vi "UMLEditor Main.vi"(1 "StartProject":string, 3 "StartTarget":string) -> ()   [LabVIEW 2020] (continued)
            n1299 = call <resource>:"CommonVIs SterotypeStringParser.vi"("SterotypeStringIn"=w3426) -> ("Name"=w3422:string)  [unwired: 18 out]
            n1300 = Search 1D Array(1D array=w3423, element=w3422) -> (index of element=w3421:i32)  [unwired: 1 out]
            n1301 = Less Than 0?(x=w3421) -> (x < 0?=w3418:bool)
            n1302 = case shown="False" w3418 {
              selector: w3418 -> [_ w3466]
              tunnel: [w3462 w3466] -> w3417
              frame False {
                n1303 = Two Button Dialog(message="There is already on object on the diagram with this name.\nDo you want to add this object anyway?" ("regular expression"), 1:"Cancel" ("regular expression"), 2:"Add object" ("regular expression")) -> (T button?=w3462:bool)
              }
              frame True {
              }
            }
            n1304 = Compound Arithmetic op=AND(TRUE, w3437, w3435, w3417) -> (w3436:bool)
            n1305 = case shown="False" w3436 {
              tunnel: w3461 -> [w3478 w3515]
              tunnel: [w3478 w3514] -> w3460
              tunnel: w3424 -> [w3470 w3513]
              tunnel: w3427 -> [w3471 w3512]
              tunnel: [w3477 w3507] -> w3458
              tunnel: [w3469 w3506] -> w3457
              tunnel: w3426 -> [_ w3505]
              tunnel: w3453 -> [w3467 w3504]
              tunnel: w3451 -> [_ w3502]
              tunnel: w3428 -> [_ w3503]
              tunnel: w3420 -> [w3476 _]
              tunnel: w3419 -> [w3468 _]
              frame False {
                n1306 = call <vilib>:"Check if File or Folder Exists.vi"("path"=w3467) -> ("file or folder exists?"=w3473:bool)  [unwired: 1 in, 9 out]
                n1307 = Equal?(x=T27 "StateDiagramGraph" ("diagramType"), y=w3476) -> (x = y?=w3474:bool)
                n1308 = And(x=w3474, y=w3473) -> (x .and. y?=w3472:bool)
                n1309 = case shown="True" w3472 {
                  tunnel: [UMLEditor_statesType."Idle" ("state") UMLEditor_statesType."Repaint" ("state")] -> w3477
                  tunnel: w3471 -> [_ w3485]
                  tunnel: w3470 -> [w3479 w3483]
                  tunnel: [w3479 w3491] -> w3469
                  tunnel: w3468 -> [_ w3489]
                  tunnel: w3467 -> [_ w3486]
                  frame False {
                  }
                  frame True {
                    n1310 = To More Specific Class(target class=refnum<class "StateDiagramGraph.lvclass"> refnum ("reference out"), reference=w3485, error in=w3483) -> (specific class reference=w3484:refnum<class "StateDiagramGraph.lvclass">, error out=w3482:errorcluster)
                    n1311 = Unbundle By Name(w3489) -> ("graphics"=w3488:refnum<class "Graphics.lvclass">, "grid"=w3487:refnum<class "Grid.lvclass">)
                    n1312 = call <resource>:"SetPathInfo.vi"("reference"=w3484, "StateDiagramData.VI-Path"=w3486, "error in (no error)"=w3482) -> ("reference out"=w3493:refnum<class "StateDiagramGraph.lvclass">, "error out"=w3492:errorcluster)  [unwired: 1 in, 14 out]
                    n1313 = call-dynamic "HandleRightClickMenuOption.vi"("reference"=w3493, "MenuOption"="Update diagram...", "graphics"=w3488, "grid"=w3487, "error in (no error)"=w3492) -> ("error out"=w3491:errorcluster)  [unwired: 12 in, 2 out]
                  }
                }
              }
              frame True {
                n1314 = call-dynamic "findNode.vi"("reference"=w3512, "error in (no error)"=w3513) -> ("reference out"=w3499:refnum<class "Graph.lvclass">, "node"=w3511:refnum<class "AbstractNode.lvclass">, "found"=w3510:bool, "error out"=w3497:errorcluster)  [unwired: 14 in]
                n1315 = call <resource>:"ClassNode_Create.vi"("error in (no error)"=w3497) -> ("reference out"=w3495:refnum<class "ClassNode.lvclass">, "error out"=w3496:errorcluster)  [unwired: 17 in]
                n1316 = call <resource>:"FindFreePosition.vi"("reference"=w3499, "NodePointIn"=w3502, "Node"=w3495, "error in (no error)"=w3496) -> ("reference out"=w3498:refnum<class "Graph.lvclass">, "NodePointOut"=w3501:T9, "error out"=w3500:errorcluster)  [unwired: 13 out]
                n1317 = call-dynamic "add.vi"("reference"=w3498, "node"=w3495, "point"=w3501, "error in (no error)"=w3500) -> ("added"=w3509:bool, "error out"=w3508:errorcluster)  [unwired: 13 in, 1 out]
                n1318 = case shown="True" w3509 {
                  tunnel: w3515 -> [w3525 w3556]
                  tunnel: [w3524 w3554] -> w3514
                  tunnel: w3508 -> [w3520 w3551]
                  tunnel: w3495 -> [w3518 w3540]
                  tunnel: w3501 -> [w3522 w3552]
                  tunnel: [w3521 w3557] -> w3506
                  tunnel: w3510 -> [w3517 _]
                  tunnel: w3511 -> [w3523 _]
                  tunnel: w3505 -> [_ w3549]
                  tunnel: [UMLEditor_statesType."Idle" ("state") w3548] -> w3507
                  tunnel: w3504 -> [_ w3542]
                  tunnel: w3503 -> [_ w3541]
                  frame False {
                    n1319 = call-dynamic "Destroy.vi"("reference"=w3518, "error in (no error)"=w3520) -> ("error out"=w3519:errorcluster)  [unwired: 16 in, 1 out]
                    n1320 = case shown="True" w3517 {
                      tunnel: w3525 -> [w3526 w3539]
                      tunnel: [w3526 w3538] -> w3524
                      tunnel: w3523 -> [_ w3537]
                      tunnel: w3522 -> [_ w3536]
                      tunnel: [w3527 w3535] -> w3521
                      tunnel: w3519 -> [w3527 w3534]
                      frame False {
                      }
                      frame True {
                        # "Node Found"
                        n1321 = call-dynamic "getBounds.vi"("reference"=w3537, "error in (no error)"=w3534) -> ("bounds"=w3532:T10, "error out"=w3535:errorcluster)  [unwired: 15 in, 1 out]
                        n1322 = Build Array(w3537) -> (w3531:refnum<class "AbstractNode.lvclass">[])
                        n1323 = Bundle By Name(cluster=w3539, "selected"=UMLEditor_tooltype."Node" ("selcted"), "SelectedNodes"=w3531, "dragStartBounds"=w3532, "dragStartPoint"=w3536, "lastMousePoint"=w3536, "newSelected"=TRUE, "toolType"=UMLEditor_tooltype."None") -> (w3538:T5)
                        n1324 = local write "GraphButtons"(T1."1" ("GraphButtons")) -> ()
                      }
                    }
                  }
                  frame True {
                    # "Added"
                    n1325 = case shown="\"AddNodeFromProjectTree+SyncAll\"" w3541 {
                      tunnel: [UMLEditor_statesType."Repaint" ("state") UMLEditor_statesType."SyncAll" ("state")] -> w3548
                      frame "AddNodeFromProjectTree", Default {
                      }
                      frame "AddNodeFromProjectTree+SyncAll" {
                      }
                    }
                    n1326 = call-dynamic "ExternalSetParam.vi"("reference"=w3540, "setParameter"=ExternalSetTypes."Name", "string"=w3549, "error in (no error)"=w3551) -> ("reference out"=w3545:refnum<class "ClassNode.lvclass">, "error out"=w3547:errorcluster)  [unwired: 14 in]
                    n1327 = call-dynamic "ExternalSetParam.vi"("reference"=w3545, "setParameter"=ExternalSetTypes."ClassPath", "error in (no error)"=w3547, "ClassPath"=w3542) -> ("reference out"=w3544:refnum<class "ClassNode.lvclass">, "error out"=w3546:errorcluster)  [unwired: 14 in]
                    n1328 = call-dynamic "getBounds.vi"("reference"=w3544, "error in (no error)"=w3546) -> ("reference out"=w3561:refnum<class "ClassNode.lvclass">, "bounds"=w3562:T10, "error out"=w3558:errorcluster)  [unwired: 15 in]
                    n1329 = Build Array(w3561) -> (w3553:refnum<class "ClassNode.lvclass">[])
                    n1330 = Bundle By Name(cluster=w3556, "selected"=UMLEditor_tooltype."Node" ("selcted"), "SelectedNodes"=w3553, "dragStartBounds"=w3562, "dragStartPoint"=w3552, "lastMousePoint"=w3552) -> (w3555:T5)
                    n1331 = call <resource>:"UMLEditor setDiagramInfo.vi"("error in (no error)"=w3558, "localVariablesIn"=w3555, "action"=enum16{"Name/Dir", "Unsaved", "Saved"}."Unsaved") -> ("localVariablesOut"=w3554:T5, "error out"=w3557:errorcluster)  [unwired: 2 in, 13 out]
                  }
                }
              }
            }
            n1332 = for {
              tunnel: w3457 -> [_]
              tunnel: w3432 -> [w3577] mode=indexing
              tunnel: [w3576] -> _
              n1333 = Close Reference(reference=w3577) -> (error out=w3576:errorcluster)  [unwired: 1 in]
            }
          }
          frame True {
            n1334 = call <resource>:"GDSError_ClearError.vi"("code"=1055, "error in (no error)"=w3580) -> ("error out"=w3579:errorcluster)  [unwired: 3 in, 14 out]
          }
        }
      }
      frame "AnalyseViInStateDiagram" {
        n1335 = Unbundle By Name(w3589) -> ("diagrams"=w3610:T8[])
        n1336 = Unbundle By Name(w3589) -> ("menu"=w3604:refnum<k9>, "Action"=w3588:string)
        n1337 = property on="GraphButtons" class="RadioBtnsControl (strict)"("Disabled"=u8 0) -> ()  [unwired: 2 in, 2 out]
        n1338 = local write "Diagram"(0) -> ()
        n1339 = local write "GraphButtons"(T1."1" ("GraphButtons")) -> ()
        n1340 = for {
          tunnel: w3610 -> [w3654] mode=indexing
          tunnel: "Untitled %d" -> [w3652]
          tunnel: [w3651] -> w3608 mode=indexing
          n1341 = Unbundle By Name(w3654) -> ("name"=w3653:string)
          n1342 = Scan From String(format string=w3652, input string=w3653) -> (output 1=w3651:i32)  [unwired: 2 in, 4 out]
        }
        n1343 = String To Path(string=w3588) -> (path=w3587:path)
        n1344 = Bundle By Name(cluster=T29 {"VI-Path"=path "", "ShowOption"=enum."Show Relative Path"} ("StateDiagramData"), "VI-Path"=w3587) -> (w3594:T29)
        n1345 = Unbundle By Name(w3589) -> ("grid"=w3596:refnum<class "Grid.lvclass">, "graphics"=w3595:refnum<class "Graphics.lvclass">)
        n1346 = Array Max & Min(array=w3608) -> (max value=w3607:i32)  [unwired: 3 out]
        n1347 = call <resource>:"StateDiagramGraph_Create.vi"("StateDiagramData"=w3594, "error in (no error)"=w3593) -> ("reference out"=w3599:refnum<class "StateDiagramGraph.lvclass">, "error out"=w3598:errorcluster)  [unwired: 1 in, 15 out]
        n1348 = property on="Picture" class="Pict"() -> (error out=w3586:errorcluster, "Visible"=w3585:bool)  [unwired: 2 in, 1 out]
        n1349 = call-dynamic "HandleRightClickMenuOption.vi"("reference"=w3599, "MenuOption"="Create New Diagram", "graphics"=w3595, "grid"=w3596, "error in (no error)"=w3598) -> ("reference out"=w3592:refnum<class "StateDiagramGraph.lvclass">, "Cancel"=w3591:bool, "error out"=w3590:errorcluster)  [unwired: 12 in]
        n1350 = property on="Picture" class="Pict"(error in=w3586, "Visible"=TRUE) -> ()  [unwired: 1 in, 2 out]
        n1351 = case shown="False" w3591 {
          tunnel: w3607 -> [w3636 _]
          tunnel: w3604 -> [w3623 _]
          tunnel: [w3622 w3648] -> w3603
          tunnel: [w3621 w3647] -> w3602
          tunnel: w3589 -> [w3620 w3647]
          tunnel: [UMLEditor_statesType."Repaint" ("state") UMLEditor_statesType."Idle" ("state")] -> w3601
          tunnel: w3592 -> [w3618 w3649]
          tunnel: w3590 -> [w3617 w3650]
          tunnel: w3585 -> [_ w3645]
          frame False {
            n1352 = local read "Help"() -> (w3613:bool)
            n1353 = call <resource>:"UndoEngine.vi"("Reference In"=w3618, "Action"=enum16{"TakeSnapshot", "Undo", "Redo"}."TakeSnapshot", "Reset"=TRUE, "error in (no error)"=w3617, "menu"=w3623) -> ("Reference Out"=w3615:refnum<class "StateDiagramGraph.lvclass">, "error out"=w3612:errorcluster)  [unwired: 3 in, 10 out]
            n1354 = case shown="True" w3613 {
              tunnel: w3615 -> [w3639 w3644]
              tunnel: [w3639 w3643] -> w3614
              tunnel: [w3638 w3642] -> w3611
              tunnel: w3612 -> [w3638 w3641]
              frame False {
              }
              frame True {
                n1355 = call-dynamic "GetDiagramHelpText.vi"("reference in"=w3644, "error in (no error)"=w3641) -> ("reference out"=w3643:refnum<class "StateDiagramGraph.lvclass">, "HelpOut"=w3640:T38, "error out"=w3642:errorcluster)  [unwired: 15 in]
                n1356 = call <resource>:"ContextHelp_SendMessageToPopUp.vi"("PopUpMessage"=w3640) -> ()  [unwired: 2 in, 17 out]
              }
            }
            n1357 = Increment(x=w3636) -> (x+1=w3634:i32)
            n1358 = Format Into String(format string="Untitled %d", w3634) -> (resulting string=w3631:string)  [unwired: 2 in, 1 out]
            n1359 = property on="Diagram" class="Ring (strict)"("Tip Strip"=w3631) -> ()  [unwired: 2 in, 2 out]
            n1360 = call <resource>:"UMLEditor addDiagram.vi"("graph"=w3614, "name"=w3631, "saveDir"=path "", "unsaved(False)"=FALSE, "error in (no error)"=w3611, "localVariablesIn"=w3620) -> ("localVariablesOut"=w3616:T5, "error out"=w3632:errorcluster)  [unwired: 1 in, 11 out]
            n1361 = Unbundle By Name(w3620) -> ("menu"=w3629:refnum<k9>)
            n1362 = Bundle By Name(cluster=w3616, "selectedEdge"=refnum<class "AbstractEdge.lvclass"> refnum, "SelectedNodes"=refnum<class "AbstractNode.lvclass">[] [], "selected"=UMLEditor_tooltype."None" ("selcted")) -> (w3621:T5)
            n1363 = call <resource>:"UMLEditor menuUpdates.vi"("menu"=w3629, "menuAction"=UMLEditor_MenuActionType."EnableSave", "error in (no error)"=w3632) -> ("error out"=w3622:errorcluster)  [unwired: 3 in, 13 out]
          }
          frame True {
            n1364 = property on="Picture" class="Pict"("Visible"=w3645) -> ()  [unwired: 2 in, 2 out]
            n1365 = call-dynamic "Destroy.vi"("reference"=w3649, "error in (no error)"=w3650) -> ("error out"=w3648:errorcluster)  [unwired: 17 in]
          }
        }
      }
      frame "Copy", "CopyPaste" {
        n1366 = Unbundle By Name(w3656) -> ("SelectedNodes"=w3657:refnum<class "AbstractNode.lvclass">[], "menu"=w3660:refnum<k9>)
        n1367 = Array Size(array=w3657) -> (size(s)=w3661:i32)
        n1368 = case shown="1.." w3661 {
          tunnel: w3660 -> [_ w3677]
          tunnel: w3659 -> [w3665 w3669]
          tunnel: [w3665 w3670] -> w3658
          tunnel: w3657 -> [_ w3671]
          tunnel: w3656 -> [_ w3666]
          frame 0, Default {
          }
          frame 1.. {
            n1369 = call <resource>:"UMLEditor getDiagramInfo.vi"("localVariables"=w3666, "error in (no error)"=w3669) -> ("graph"=w3667:refnum<class "Graph.lvclass">, "error out"=w3668:errorcluster)  [unwired: 16 out]
            n1370 = call <resource>:"UMLEditor menuUpdates.vi"("menu"=w3677, "menuAction"=UMLEditor_MenuActionType."EnablePaste", "error in (no error)"=w3668) -> ("error out"=w3675:errorcluster)  [unwired: 3 in, 13 out]
            n1371 = call <resource>:"UMLEditor ClipBoard.vi"("menuAction"=UMLEditor_ClipBoardActionType."EmptyClipBoard", "error in (no error)"=w3675) -> ("error out"=w3673:errorcluster)  [unwired: 4 in, 13 out]
            n1372 = call <resource>:"UMLEditor ClipBoard.vi"("menuAction"=UMLEditor_ClipBoardActionType."InsertToClipBoard", "SelectedNodes"=w3671, "Graph"=w3667, "error in (no error)"=w3673) -> ("error out"=w3670:errorcluster)  [unwired: 2 in, 13 out]
          }
        }
        n1373 = case shown="\"CopyPaste\"" w3655 {
          tunnel: [UMLEditor_statesType."Paste" ("state") UMLEditor_statesType."Idle" ("state")] -> w3662
          frame "CopyPaste" {
          }
          frame Default {
          }
        }
      }
      frame "Paste" {
        n1374 = Unbundle By Name(w3679) -> ("graphics"=w3684:refnum<class "Graphics.lvclass">, "offset"=w3686:T9, "zoom"=w3685:dbl)
        n1375 = call <resource>:"UMLEditor getDiagramInfo.vi"("localVariables"=w3679, "error in (no error)"=w3683) -> ("graph"=w3680:refnum<class "Graph.lvclass">, "diagramType"=w3681:T27, "error out"=w3682:errorcluster)  [unwired: 15 out]
        n1376 = case shown="Default" w3681 {
          tunnel: [w3690 w3712] -> w3687
          tunnel: w3686 -> [_ w3709]
          tunnel: w3685 -> [_ w3708]
          tunnel: w3684 -> [_ w3707]
          tunnel: w3682 -> [w3690 w3699]
          tunnel: w3680 -> [_ w3698]
          tunnel: w3679 -> [w3689 w3697]
          tunnel: [w3689 w3696] -> w3678
          frame "", "None" {
          }
          frame Default {
            w3706 = cluster{dbl, dbl} {0.0, 0.0} ("lower limit")
            n1377 = property on="Picture" class="Pict"() -> ("Mouse"=w3701:T41)  [unwired: 2 in, 2 out]
            n1378 = Unbundle By Name(w3701) -> ("Mouse Position"=w3711:cluster{"X":i32, "Y":i32})
            n1379 = Add(x=w3711, y=w3709) -> (x+y=w3710:T9)
            n1380 = Divide(x=w3710, y=w3708) -> (x/y=w3692:T9)
            n1381 = call <resource>:"getScreenBounds.vi"("reference"=w3707, "error in (no error)"=w3699) -> ("bounds"=w3705:T10, "error out"=w3700:errorcluster)  [unwired: 16 out]
            n1382 = Unbundle By Name(w3705) -> ("width"=w3704:dbl, "height"=w3703:dbl)
            n1383 = Bundle(cluster=w3706, w3704, w3703) -> ()  [unwired: 1 out]
            n1384 = In Range and Coerce(upper limit=w3692, x=w3692, lower limit=w3706) -> (coerced(x)=w3702:T9)  [unwired: 1 out]
            n1385 = call <resource>:"UMLEditor ClipBoard.vi"("menuAction"=UMLEditor_ClipBoardActionType."PasteContentAtPos", "Pos"=w3702, "Graph"=w3698, "error in (no error)"=w3700, "LimitPasteToAllowedLocations(True)"=FALSE) -> ("PastedNodes"=w3695:refnum<class "AbstractNode.lvclass">[], "error out"=w3712:errorcluster)  [unwired: 2 in, 11 out]
            n1386 = Array Size(array=w3695) -> (size(s)=w3693:i32)
            n1387 = case shown="0" w3693 {
              tunnel: [UMLEditor_tooltype."Node" ("selcted") UMLEditor_tooltype."None" ("selcted")] -> w3694
              frame Default {
              }
              frame 0 {
              }
            }
            n1388 = Bundle By Name(cluster=w3697, "selected"=w3694, "SelectedNodes"=w3695) -> (w3696:T5)
          }
        }
      }
      frame "Export" {
        w3717 = 0.0 ("y")
        w3716 = 5.0  # borderRoundPicture
        w3751 = 1.0 ("scaleX")
        n1389 = Unbundle By Name(w3724) -> ("graphics"=w3754:refnum<class "Graphics.lvclass">)
        n1390 = Unbundle By Name(w3724) -> ("exportype"=w3723:T11)
        n1391 = Unbundle By Name(w3724) -> ("grid"=w3746:refnum<class "Grid.lvclass">)
        n1392 = call-dynamic "clone.vi"("reference"=w3754, "error in (no error)"=w3753) -> ("clonedObjectRef"=w3752:refnum<class "Graphics.lvclass">, "error out"=w3750:errorcluster)  [unwired: 15 in, 1 out]
        n1393 = call <resource>:"scale.vi"("reference"=w3752, "scaleX"=w3751, "scaleY"=w3751, "error in (no error)"=w3750) -> ("reference out"=w3742:refnum<class "Graphics.lvclass">, "error out"=w3743:errorcluster)  [unwired: 14 out]
        n1394 = call <resource>:"resetPicture.vi"("reference"=w3742, "error in (no error)"=w3743) -> ("reference out"=w3741:refnum<class "Graphics.lvclass">, "error out"=w3740:errorcluster)  [unwired: 16 out]
        n1395 = call <resource>:"UMLEditor getDiagramInfo.vi"("localVariables"=w3724, "error in (no error)"=w3740) -> ("graph"=w3748:refnum<class "Graph.lvclass">, "name"=w3721:string, "saveDir"=w3722:path, "error out"=w3749:errorcluster)  [unwired: 14 out]
        n1396 = call-dynamic "getBounds.vi"("reference"=w3748, "graphics"=w3741, "error in (no error)"=w3749) -> ("reference out"=w3747:refnum<class "Graph.lvclass">, "bounds"=w3734:T10, "error out"=w3739:errorcluster)  [unwired: 14 in]
        n1397 = Unbundle By Name(w3734) -> ("width"=w3732:dbl, "height"=w3733:dbl)
        n1398 = Unbundle By Name(w3734) -> ("x"=w3738:dbl, "y"=w3735:dbl)
        n1399 = Subtract(x=w3738, y=w3717) -> (x-y=w3737:dbl)
        n1400 = Subtract(x=w3735, y=w3717) -> (x-y=w3736:dbl)
        n1401 = Add(x=w3732, y=w3733) -> (x+y=w3731:dbl)
        n1402 = Greater Than 0?(x=w3731) -> (x > 0?=w3730:bool)
        n1403 = call <resource>:"setOffset.vi"("reference"=w3741, "offsetX"=w3737, "offsetY"=w3736, "error in (no error)"=w3739) -> ("reference out"=w3729:refnum<class "Graphics.lvclass">, "error out"=w3718:errorcluster)  [unwired: 14 out]
        n1404 = Multiply(x=w3716, y=2.0) -> (x*y=w3725:dbl)
        n1405 = call-dynamic "draw.vi"("reference"=w3747, "graphics"=w3729, "grid"=w3746, "error in (no error)"=w3718, "SelectedNodes"=refnum<class "AbstractNode.lvclass">[] [], "HideOverLays(False)"=TRUE) -> ("NodesBounds"=w3745:T10, "error out"=w3727:errorcluster)  [unwired: 10 in, 2 out]
        n1406 = case shown="True" w3730 {
          tunnel: w3745 -> [_ _]
          tunnel: w3734 -> [_ w3778]
          tunnel: w3729 -> [_ w3779]
          tunnel: w3727 -> [w3756 w3764]
          tunnel: [w3756 w3764] -> w3728
          tunnel: w3725 -> [_ w3768]
          tunnel: w3723 -> [_ w3763]
          tunnel: w3723 -> [_ w3771]
          tunnel: w3722 -> [_ w3770]
          tunnel: w3721 -> [_ w3765]
          tunnel: w3716 -> [_ w3758]
          frame False {
          }
          frame True {
            n1407 = Match Pattern(string=w3765, regular expression="[.][~.]+$") -> (before substring=w3766:string)  [unwired: 4 out]
            n1408 = Unbundle By Name(w3778) -> ("x"=w3761:dbl, "y"=w3759:dbl, "width"=w3776:dbl, "height"=w3774:dbl)
            n1409 = case shown="\"jpg\"" w3771 {
              tunnel: w3770 -> [_ w3787 w3792 _]
              tunnel: w3766 -> [_ w3785 w3790 _]
              tunnel: [path "" ("Not A Path Constant") w3783 w3788 path "" ("Not A Path Constant")] -> w3769
              frame "None", Default {
              }
              frame "png" {
                n1410 = Concatenate Strings(w3785, ".png" ("string")) -> (w3786:string)
                n1411 = Build Path(base path=w3787, name or relative path=w3786) -> (appended path=w3783:path)
              }
              frame "jpg" {
                n1412 = Concatenate Strings(w3790, ".jpg" ("string")) -> (w3791:string)
                n1413 = Build Path(base path=w3792, name or relative path=w3791) -> (appended path=w3788:path)
              }
              frame "Printer" {
              }
            }
            n1414 = Subtract(x=w3761, y=w3758) -> (x-y=w3760:dbl)
            n1415 = Subtract(x=w3759, y=w3758) -> (x-y=w3757:dbl)
            n1416 = Add(x=w3776, y=w3768) -> (x+y=w3775:dbl)
            n1417 = Add(x=w3774, y=w3768) -> (x+y=w3773:dbl)
            n1418 = Bundle By Name(cluster=T10 {"x"=0.0, "y"=0.0, "width"=0.0, "height"=0.0} ("bounds"), "x"=w3760, "y"=w3757, "width"=w3775, "height"=w3773) -> (w3772:T10)
            n1419 = call <resource>:"UMLEditor export.vi"("graphics"=w3779, "bounds"=w3772, "exportype"=w3763, "fileName"=w3769, "error in (no error)"=w3764) -> ("error out"=w3762:errorcluster)  [unwired: 14 out]
            n1420 = case shown="\"Printer\"" w3763 {
              tunnel: w3762 -> [_ w3780]
              frame "None", Default {
              }
              frame "Printer" {
                n1421 = case shown="Error" w3780 {
                  frame No Error {
                  }
                  frame Error {
                    n1422 = One Button Dialog(message="Error while printing\nCheck the default printer settings.") -> ()  [unwired: 2 out]
                  }
                }
              }
            }
          }
        }
        n1423 = call-dynamic "Destroy.vi"("reference"=w3729, "error in (no error)"=w3728) -> ("error out"=w3744:errorcluster)  [unwired: 16 in, 1 out]
      }
      frame "EditSelected" {
        n1424 = Unbundle By Name(w3796) -> ("selected"=w3807:T7, "selectedEdge"=w3801:refnum<class "AbstractEdge.lvclass">, "SelectedNodes"=w3805:refnum<class "AbstractNode.lvclass">[])
        n1425 = Unbundle By Name(w3796) -> ("graphics"=w3795:refnum<class "Graphics.lvclass">, "grid"=w3794:refnum<class "Grid.lvclass">)
        n1426 = call <resource>:"UMLEditor getDiagramInfo.vi"("localVariables"=w3796, "error in (no error)"=w3804) -> ("graph"=w3802:refnum<class "Graph.lvclass">, "diagramType"=w3799:T27, "error out"=w3803:errorcluster)  [unwired: 15 out]
        n1427 = Bundle By Name(cluster=w3796, "newSelected"=FALSE) -> (w3798:T5)
        n1428 = case shown="\"Node\"" w3807 {
          tunnel: w3803 -> [w3813 w3843 w3911]
          tunnel: [w3811 w3844 w3905] -> w3806
          tunnel: w3805 -> [_ w3832 _]
          tunnel: w3802 -> [w3812 w3839 w3909]
          tunnel: w3801 -> [_ _ w3908]
          tunnel: w3798 -> [w3810 w3830 w3907]
          tunnel: [w3809 w3834 w3906] -> w3800
          tunnel: w3799 -> [w3814 _ _]
          tunnel: w3795 -> [_ w3827 _]
          tunnel: w3794 -> [_ w3826 _]
          frame "None", Default {
            n1429 = case shown="\"StateDiagramGraph\"" w3814 {
              tunnel: w3813 -> [w3816 w3825]
              tunnel: w3812 -> [_ w3819]
              tunnel: [w3816 w3822] -> w3811
              tunnel: w3810 -> [w3815 w3821]
              tunnel: [w3815 w3820] -> w3809
              frame Default {
              }
              frame "StateDiagramGraph" {
                n1430 = To More Specific Class(target class=refnum<class "StateDiagramGraph.lvclass"> refnum ("reference out"), reference=w3819) -> (specific class reference=w3817:refnum<class "StateDiagramGraph.lvclass">)  [unwired: 1 in, 1 out]
                n1431 = call-dynamic "editDialog.vi"("reference"=w3817, "error in (no error)"=w3825) -> ("error out"=w3823:errorcluster)  [unwired: 15 in, 2 out]
                n1432 = call <resource>:"UMLEditor setDiagramInfo.vi"("error in (no error)"=w3823, "localVariablesIn"=w3821, "action"=enum16{"Name/Dir", "Unsaved", "Saved"}."Unsaved") -> ("localVariablesOut"=w3820:T5, "error out"=w3822:errorcluster)  [unwired: 2 in, 13 out]
              }
            }
          }
          frame "Node" {
            n1433 = Index Array(array=w3832) -> (element=w3829:refnum<class "AbstractNode.lvclass">)  [unwired: 1 in]
            n1434 = call-dynamic "contains.vi"("reference"=w3839, "node"=w3829, "nodeType(Empty=AllNodeTypesAllaowed)"=string[] ["PackageNode$", "SystemNode$"], "error in (no error)"=w3843) -> ("contains"=w3838:bool, "container"=w3837:refnum<class "AbstractNode.lvclass">, "error out"=w3842:errorcluster)  [unwired: 12 in, 1 out]
            n1435 = call-dynamic "editDialog.vi"("reference"=w3829, "insidePackageNode"=w3838, "error in (no error)"=w3842) -> ("reference out"=w3836:refnum<class "AbstractNode.lvclass">, "changeConnection"=w3841:T54, "cancel"=w3835:bool, "error out"=w3840:errorcluster)  [unwired: 13 in]
            n1436 = Build Array(w3829) -> (w3828:refnum<class "AbstractNode.lvclass">[])
            n1437 = Bundle By Name(cluster=w3830, "SelectedNodes"=w3828) -> (w3831:T5)
            n1438 = case shown="False" w3835 {
              tunnel: [w3851 w3903] -> w3844
              tunnel: w3841 -> [w3858 _]
              tunnel: w3840 -> [w3857 w3903]
              tunnel: w3839 -> [w3847 _]
              tunnel: w3837 -> [w3856 _]
              tunnel: w3836 -> [w3855 _]
              tunnel: w3831 -> [w3850 w3902]
              tunnel: [w3849 w3902] -> w3834
              tunnel: w3827 -> [w3846 _]
              tunnel: w3826 -> [w3845 _]
              frame False {
                n1439 = case shown="\"Connect\"" w3858 {
                  tunnel: w3857 -> [w3861 w3869 w3874]
                  tunnel: w3856 -> [_ w3868 w3895]
                  tunnel: w3855 -> [w3860 w3866 w3872]
                  tunnel: [w3861 w3863 w3886] -> w3854
                  tunnel: [w3859 _ _] -> w3848
                  tunnel: w3847 -> [_ w3862 w3890]
                  tunnel: w3846 -> [_ _ w3889]
                  tunnel: w3845 -> [_ _ w3888]
                  frame "NA", Default {
                    n1440 = Build Array(w3860) -> (w3859:refnum<class "AbstractNode.lvclass">[])
                  }
                  frame "Connect" {
                    n1441 = call-dynamic "addChild.vi"("reference"=w3868, "node"=w3866, "error in (no error)"=w3869) -> ("reference out"=w3865:refnum<class "AbstractNode.lvclass">, "error out"=w3867:errorcluster)  [unwired: 15 in]
                    n1442 = call-dynamic "setParent.vi"("reference"=w3866, "node"=w3865, "error in (no error)"=w3867) -> ("error out"=w3864:errorcluster)  [unwired: 15 in, 1 out]
                    n1443 = call-dynamic "RearrangeNodes.vi"("reference in"=w3862, "error in (no error)"=w3864) -> ("error out"=w3863:errorcluster)  [unwired: 16 in, 1 out]
                  }
                  frame "DisConnect" {
                    n1444 = call-dynamic "GetParentsRecurivly.vi"("reference"=w3872, "error in (no error)"=w3874) -> ("Parents"=w3871:refnum<class "AbstractNode.lvclass">[], "error out"=w3873:errorcluster)  [unwired: 15 in, 1 out]
                    n1445 = call-dynamic "removeChild.vi"("reference"=w3895, "node"=w3872, "error in (no error)"=w3873) -> ("reference out"=w3891:refnum<class "AbstractNode.lvclass">, "error out"=w3894:errorcluster)  [unwired: 15 in]
                    n1446 = call-dynamic "setParent.vi"("reference"=w3872, "node"=refnum<class "AbstractNode.lvclass"> refnum, "error in (no error)"=w3894) -> ("error out"=w3892:errorcluster)  [unwired: 15 in, 1 out]
                    n1447 = call-dynamic "layout.vi"("reference"=w3891, "graph"=w3890, "graphics"=w3889, "grid"=w3888, "error in (no error)"=w3892) -> ("error out"=w3887:errorcluster)  [unwired: 13 in, 1 out]
                    n1448 = Delete From Array(array=w3871) -> (deleted portion=w3870:refnum<class "AbstractNode.lvclass">)  [unwired: 2 in, 1 out]
                    n1449 = call-dynamic "getBounds.vi"("reference"=w3870, "error in (no error)"=w3887) -> ("bounds"=w3884:T10, "error out"=w3885:errorcluster)  [unwired: 15 in, 1 out]
                    n1450 = call <resource>:"Rectangel GetRectInfo.vi"("bounds"=w3884) -> ("maxX"=w3882:dbl)  [unwired: 1 in, 17 out]
                    n1451 = call-dynamic "getBounds.vi"("reference"=w3872, "error in (no error)"=w3885) -> ("reference out"=w3877:refnum<class "AbstractNode.lvclass">, "bounds"=w3883:T10, "error out"=w3876:errorcluster)  [unwired: 15 in]
                    n1452 = Unbundle By Name(w3883) -> ("x"=w3881:dbl)
                    n1453 = Subtract(x=w3882, y=w3881) -> (x-y=w3880:dbl)
                    n1454 = Add(x=10.0, y=w3880) -> (x+y=w3878:dbl)
                    n1455 = Greater Or Equal To 0?(x=w3878) -> (x >= 0?=w3875:bool)
                    n1456 = case shown="True" w3875 {
                      tunnel: [w3896 w3901] -> w3886
                      tunnel: w3878 -> [_ w3900]
                      tunnel: w3877 -> [_ w3899]
                      tunnel: w3876 -> [w3896 w3898]
                      frame False {
                      }
                      frame True {
                        n1457 = call-dynamic "translate.vi"("reference"=w3899, "dx"=w3900, "dy"=0.0, "error in (no error)"=w3898) -> ("error out"=w3901:errorcluster)  [unwired: 14 in, 1 out]
                      }
                    }
                  }
                }
                n1458 = call-dynamic "layout.vi"("reference"=w3847, "LayoutNodes(Empty=All)"=w3848, "error in (no error)"=w3854) -> ("error out"=w3852:errorcluster)  [unwired: 15 in, 1 out]
                n1459 = call <resource>:"UMLEditor setDiagramInfo.vi"("error in (no error)"=w3852, "localVariablesIn"=w3850, "action"=enum16{"Name/Dir", "Unsaved", "Saved"}."Unsaved") -> ("localVariablesOut"=w3849:T5, "error out"=w3851:errorcluster)  [unwired: 2 in, 13 out]
              }
              frame True {
              }
            }
          }
          frame "Edge" {
            n1460 = call-dynamic "editDialog.vi"("reference"=w3908, "error in (no error)"=w3911) -> ("cancel"=w3904:bool, "error out"=w3910:errorcluster)  [unwired: 15 in, 1 out]
            n1461 = case shown="True" w3904 {
              tunnel: w3910 -> [w3919 w3925]
              tunnel: w3909 -> [w3918 _]
              tunnel: w3907 -> [w3916 w3924]
              tunnel: [w3915 w3924] -> w3906
              tunnel: [w3913 w3925] -> w3905
              frame False {
                n1462 = case shown="False" FALSE ("Case Constant\n(See Context Help) 4") {
                  tunnel: w3919 -> [w3920 w3923]
                  tunnel: w3918 -> [_ w3922]
                  tunnel: [w3920 w3921] -> w3914
                  frame False {
                  }
                  frame True {
                    n1463 = call-dynamic "layout.vi"("reference"=w3922, "error in (no error)"=w3923) -> ("error out"=w3921:errorcluster)  [unwired: 16 in, 1 out]
                  }
                }
                n1464 = call <resource>:"UMLEditor setDiagramInfo.vi"("error in (no error)"=w3914, "localVariablesIn"=w3916, "action"=enum16{"Name/Dir", "Unsaved", "Saved"}."Unsaved") -> ("localVariablesOut"=w3915:T5, "error out"=w3913:errorcluster)  [unwired: 2 in, 13 out]
              }
              frame True {
              }
            }
          }
        }
      }
      frame "RemoveSelected" {
        # "if aggregartion, check if we should remove ClassRef Attribute"
        n1465 = Unbundle By Name(w3934) -> ("selected"=w3930:T7, "selectedEdge"=w3936:refnum<class "AbstractEdge.lvclass">, "SelectedNodes"=w3935:refnum<class "AbstractNode.lvclass">[], "Don'tDeleteChildren"=w3926:bool)
        n1466 = call <resource>:"UMLEditor getDiagramInfo.vi"("localVariables"=w3934, "error in (no error)"=w3938) -> ("graph"=w3937:refnum<class "Graph.lvclass">, "error out"=w3927:errorcluster)  [unwired: 16 out]
        n1467 = case shown="\"Node\"" w3930 {
          tunnel: [w3951 w3959 w3979] -> w3932
          tunnel: w3937 -> [_ w3958 w3981]
          tunnel: w3927 -> [w3951 w3956 w3978]
          tunnel: w3936 -> [_ w3957 _]
          tunnel: w3935 -> [_ _ w3980]
          tunnel: w3926 -> [_ _ w3977]
          frame "None", Default {
          }
          frame "Edge" {
            n1468 = call <resource>:"UMLEditor ShowAggregationDialog.vi"("graph"=w3958, "ClassAggregation"=w3957, "error in (no error)"=w3956) -> ("Base class.bounds"=w3953:T10, "Remove"=w3954:bool, "StartEndNodes"=w3952:T37, "error out"=w3955:errorcluster)  [unwired: 13 out]
            n1469 = stacked-sequence {
              tunnel: [w3966] -> w3959
              tunnel: w3958 -> [w3965]
              tunnel: w3957 -> [w3964]
              tunnel: w3956 -> [w3963]
              tunnel: w3955 -> [_]
              tunnel: w3954 -> [w3962]
              tunnel: w3953 -> [w3961]
              tunnel: w3952 -> [w3960]
              frame #0 {
                n1470 = case shown="True" w3962 {
                  tunnel: w3961 -> [_ w3973]
                  tunnel: w3960 -> [_ w3967]
                  frame False {
                  }
                  frame True {
                    n1471 = Unbundle(w3973) -> ("x"=w3972:dbl, "y"=w3968:dbl, "width"=w3971:dbl)  [unwired: 1 out]
                    n1472 = Add(x=w3972, y=w3971) -> (x+y=w3970:dbl)
                    n1473 = Bundle(cluster=cluster{"X":i32, "Y":i32} {"X"=100, "Y"=100} ("Mouse Position"), "X"=w3970, "Y"=w3968) -> (w3969:cluster{"X":i32, "Y":i32})
                    n1474 = call <resource>:"UMLEditor_AggregationClusterDialogControl.vi"("Position"=w3969, "Action(SelectSelect)"=T19."DeleteAggregation", "StartEndNodesIn"=w3967) -> ()  [unwired: 6 in, 11 out]
                  }
                }
                n1475 = call-dynamic "removeEdge.vi"("reference"=w3965, "edge"=w3964, "error in (no error)"=w3963) -> ("error out"=w3966:errorcluster)  [unwired: 15 in, 1 out]
              }
            }
          }
          frame "Node" {
            n1476 = Not(x=w3977) -> (.not. x?=w3976:bool)
            n1477 = for {
              tunnel: w3981 -> [w3986]
              tunnel: w3980 -> [w3985] mode=indexing
              shift-right: [w3984] -> w3979
              shift-left: w3978 -> [w3983]
              tunnel: w3976 -> [w3982]
              n1478 = call-dynamic "removeNode.vi"("reference"=w3986, "node"=w3985, "RemoveChildrenIfAny(False)"=w3982, "error in (no error)"=w3983) -> ("error out"=w3984:errorcluster)  [unwired: 14 in, 1 out]
            }
          }
        }
        n1479 = Bundle By Name(cluster=w3934, "selected"=UMLEditor_tooltype."None" ("selcted")) -> (w3929:T5)
        n1480 = case shown="\"Node\", \"Edge\"" w3930 {
          tunnel: w3932 -> [w3941 w3949]
          tunnel: [w3941 w3948] -> w3931
          tunnel: [w3940 w3945] -> w3928
          tunnel: w3929 -> [w3940 w3947]
          frame "None", Default {
          }
          frame "Node", "Edge" {
            n1481 = call <resource>:"UMLEditor setDiagramInfo.vi"("error in (no error)"=w3949, "localVariablesIn"=w3947, "action"=enum16{"Name/Dir", "Unsaved", "Saved"}."Unsaved") -> ("localVariablesOut"=w3946:T5, "error out"=w3948:errorcluster)  [unwired: 2 in, 13 out]
            n1482 = Bundle By Name(cluster=w3946, "SelectedNodes"=refnum<class "AbstractNode.lvclass">[] [], "selectedEdge"=refnum<class "AbstractEdge.lvclass"> refnum, "modified"=TRUE) -> (w3945:T5)
          }
        }
      }
      frame "Save" {
        w3990 = UMLEditor_statesType."Close" ("x")
        n1483 = Unbundle By Name(w3992) -> ("saveAs"=w3994:bool)
        n1484 = call <resource>:"UMLEditor getDiagramInfo.vi"("localVariables"=w3992, "error in (no error)"=w4013) -> ("graph"=w4011:refnum<class "Graph.lvclass">, "name"=w4004:string, "saveDir"=w4001:path, "error out"=w4010:errorcluster)  [unwired: 14 out]
        n1485 = Empty String/Path?(string/path=w4001) -> (empty?=w3989:bool)
        n1486 = File/Directory Info(path=w4001, error in=w4010) -> (directory=w3999:bool, error out=w4008:errorcluster)  [unwired: 5 out]
        n1487 = call <resource>:"File_ApplicationPaths.vi"("PathName"=UMLEditor_StoredPathes."LastSearchPath" ("UMLPathes")) -> ("Path Out"=w3987:path)  [unwired: 3 in, 15 out]
        n1488 = Bundle By Name(cluster=w3992, "saveAs"=FALSE) -> (w3993:T5)
        n1489 = Compound Arithmetic op=AND(invert w3994, invert w3989, w3999) -> (w4000:bool)
        n1490 = case shown="False" w4000 {
          tunnel: w4008 -> [w4031 w4054]
          tunnel: [w4030 w4054] -> w4007
          tunnel: [w4025 w4056] -> w4006
          tunnel: w4001 -> [w4016 w4056]
          tunnel: [w4024 w4055] -> w4005
          tunnel: w4004 -> [w4023 w4055]
          tunnel: w3993 -> [w4029 w4057]
          tunnel: [w4028 w4057] -> w4003
          tunnel: [w4019 FALSE ("cancelled")] -> w4002
          tunnel: w3989 -> [w4017 _]
          tunnel: w3987 -> [w4014 _]
          frame False {
            (unwired) T49."new or existing file" ("select mode (2)")
            n1491 = Select(t=w4014, s=w4017, f=w4016) -> (s? t:f=w4015:path)
            n1492 = File Dialog(6:"*.uml" ("pattern"), 7:"Select file name" ("prompt"), 11:w4015) -> (1:w4020:bool, 2:w4022:bool, 3:w4021:path)  [unwired: 1 in, 4 out]
            n1493 = case shown="True" w4022 {
              tunnel: [w4032 w4035] -> w4019
              tunnel: w4020 -> [w4032 _]
              tunnel: w4021 -> [w4033 w4034]
              tunnel: [w4033 w4034] -> w4018
              frame False {
              }
              frame True {
                n1494 = Two Button Dialog(message="This file already exists.\nDo you want to overwrite it?", 1:"No" ("F button name (\"Cancel\")"), 2:"Yes" ("T button name (\"OK\")")) -> (T button?=w4036:bool)
                n1495 = case shown="True" w4036 {
                  tunnel: w4034 -> [_ w4040]
                  frame False {
                  }
                  frame True {
                    n1496 = Delete(path (use dialog)=w4040) -> ()  [unwired: 1 in, 6 out]
                  }
                }
                n1497 = Not(x=w4036) -> (.not. x?=w4035:bool)
              }
            }
            n1498 = case shown="False" w4019 {
              tunnel: w4031 -> [w4047 w4049]
              tunnel: [w4046 w4049] -> w4030
              tunnel: w4029 -> [w4045 w4052]
              tunnel: [w4044 w4052] -> w4028
              tunnel: w4018 -> [w4043 _]
              tunnel: [w4042 w4051] -> w4025
              tunnel: [w4041 w4050] -> w4024
              tunnel: w4015 -> [_ w4051]
              tunnel: w4023 -> [_ w4050]
              frame False {
                n1499 = Strip Path(path=w4043) -> (stripped path=w4042:path, name=w4041:string)
                n1500 = call <resource>:"UMLEditor setDiagramInfo.vi"("name"=w4041, "saveDir"=w4042, "error in (no error)"=w4047, "localVariablesIn"=w4045, "action"=enum16{"Name/Dir", "Unsaved", "Saved"}."Name/Dir") -> ("localVariablesOut"=w4044:T5, "error out"=w4046:errorcluster)  [unwired: 13 out]
              }
              frame True {
              }
            }
          }
          frame True {
          }
        }
        n1501 = Equal?(x=w3990, y=w3998) -> (x = y?=w3997:bool)
        n1502 = case shown="False" w4002 {
          tunnel: [w4061 w4089] -> w4012
          tunnel: w4011 -> [w4073 _]
          tunnel: w4007 -> [w4072 w4089]
          tunnel: w4003 -> [w4071 w4088]
          tunnel: [w4070 w4088] -> w4009
          tunnel: w4006 -> [w4066 _]
          tunnel: w4005 -> [w4069 _]
          frame False {
            n1503 = Build Path(base path=w4066, name or relative path=w4069) -> (appended path=w4065:path)
            n1504 = Path To String(path=w4065) -> (string=w4067:string)
            n1505 = call-dynamic "saveGraph.vi"("reference"=w4073, "filePath"=w4065, "error in (no error)"=w4072) -> ("reference out"=w4059:refnum<class "Graph.lvclass">, "succeeded"=w4068:bool, "error out"=w4064:errorcluster)  [unwired: 14 in]
            n1506 = property on="Diagram" class="Ring (strict)"("Tip Strip"=w4067) -> ()  [unwired: 2 in, 2 out]
            n1507 = case shown="True" w4068 {
              tunnel: w4071 -> [w4075 w4078]
              tunnel: [w4075 w4079] -> w4070
              tunnel: w4064 -> [w4076 w4086]
              tunnel: [w4076 w4084] -> w4060
              tunnel: w4065 -> [_ w4081]
              tunnel: [w4074 w4077] -> w4058
              frame False {
                n1508 = Unbundle By Name(w4075) -> ("menu"=w4074:refnum<k9>)
              }
              frame True {
                n1509 = call <resource>:"UMLEditor setDiagramInfo.vi"("error in (no error)"=w4086, "localVariablesIn"=w4078, "action"=enum16{"Name/Dir", "Unsaved", "Saved"}."Saved") -> ("localVariablesOut"=w4079:T5, "error out"=w4085:errorcluster)  [unwired: 2 in, 13 out]
                n1510 = Unbundle By Name(w4078) -> ("menu"=w4077:refnum<k9>)
                n1511 = Path To String(path=w4081) -> (string=w4082:string)
                n1512 = call <resource>:"UMLEditor menuUpdates.vi"("menu"=w4077, "menuAction"=UMLEditor_MenuActionType."AddRecentFile", "item"=w4082, "addfirst(false)"=TRUE, "error in (no error)"=w4085) -> ("error out"=w4084:errorcluster)  [unwired: 1 in, 13 out]
              }
            }
            n1513 = call <resource>:"UndoEngine.vi"("Reference In"=w4059, "Action"=enum16{"TakeSnapshot", "Undo", "Redo"}."TakeSnapshot", "Reset"=TRUE, "error in (no error)"=w4060, "menu"=w4058) -> ("error out"=w4061:errorcluster)  [unwired: 3 in, 11 out]
          }
          frame True {
          }
        }
        n1514 = Select(t=w3990, s=w3997, f=UMLEditor_statesType."Repaint" ("state")) -> (s? t:f=w3995:T6)
      }
      frame "Open" {
        n1515 = Unbundle By Name(w4098) -> ("diagrams"=w4095:T8[], "file"=w4101:path)
        n1516 = call <resource>:"UMLEditor getDiagramInfo.vi"("localVariables"=w4098, "error in (no error)"=w4115) -> ("graph"=w4114:refnum<class "Graph.lvclass">, "unsaved"=w4108:bool, "saveDir"=w4109:path, "error out"=w4112:errorcluster)  [unwired: 14 out]
        n1517 = Empty String/Path?(string/path=w4101) -> (empty?=w4102:bool)
        n1518 = Empty String/Path?(string/path=w4109) -> (empty?=w4107:bool)
        n1519 = call <resource>:"File_ApplicationPaths.vi"("PathName"=UMLEditor_StoredPathes."LastSearchPath" ("UMLPathes")) -> ("Path Out"=w4096:path)  [unwired: 3 in, 15 out]
        n1520 = case shown="True" w4102 {
          tunnel: [w4121 w4130] -> w4113
          tunnel: [w4123 w4129] -> w4111
          tunnel: w4109 -> [_ w4126]
          tunnel: w4101 -> [w4123 _]
          tunnel: "*.uml" ("pattern") -> [_ w4128]
          tunnel: w4096 -> [_ w4124]
          frame False {
            n1521 = File/Directory Info(path=w4123) -> (size=w4120:i64)  [unwired: 1 in, 6 out]
            n1522 = To Long Integer(number=w4120) -> (32bit integer=w4122:i32)
            n1523 = Greater Than 0?(x=w4122) -> (x > 0?=w4121:bool)
          }
          frame True {
            (unwired) T49."existing file" ("select mode (2)")
            n1524 = Empty String/Path?(string/path=w4126) -> (empty?=w4127:bool)
            n1525 = Select(t=w4124, s=w4127, f=w4126) -> (s? t:f=w4125:path)
            n1526 = File Dialog(6:w4128, 7:"Select file-name" ("prompt"), 11:w4125) -> (1:w4131:bool, 2:w4132:bool, 3:w4129:path)  [unwired: 1 in, 4 out]
            n1527 = Compound Arithmetic op=AND(w4132, invert w4131) -> (w4130:bool)
          }
        }
        n1528 = for {
          tunnel: w4095 -> [w4119] mode=indexing
          tunnel: [w4116] -> w4094 mode=indexing
          n1529 = Unbundle By Name(w4119) -> ("saveDir"=w4118:path, "name"=w4117:string)
          n1530 = Build Path(base path=w4118, name or relative path=w4117) -> (appended path=w4116:path)
        }
        n1531 = Compound Arithmetic op=AND(invert w4108, w4107) -> (w4106:bool)
        n1532 = Bundle By Name(cluster=w4098, "file"=path "", "Sync"=FALSE) -> (w4104:T5)
        n1533 = call <vilib>:"Set Busy.vi"("error in (no error)"=w4112) -> ("error out"=w4091:errorcluster)  [unwired: 9 in, 1 out]
        n1534 = case shown="True" w4113 {
          tunnel: w4114 -> [_ _]
          tunnel: w4091 -> [w4136 w4148]
          tunnel: w4111 -> [_ w4139]
          tunnel: w4104 -> [w4135 w4147]
          tunnel: [w4136 w4145] -> w4110
          tunnel: w4106 -> [_ w4146]
          tunnel: [w4135 w4144] -> w4105
          tunnel: [UMLEditor_statesType."Idle" ("state") w4143] -> w4100
          tunnel: w4098 -> [_ w4142]
          tunnel: w4094 -> [_ w4138]
          frame False {
          }
          frame True {
            n1535 = Unbundle By Name(w4142) -> ("graphics"=w4140:refnum<class "Graphics.lvclass">, "grid"=w4141:refnum<class "Grid.lvclass">)
            n1536 = Search 1D Array(1D array=w4138, element=w4139) -> (index of element=w4137:i32)  [unwired: 1 in]
            n1537 = case shown="-1" w4137 {
              selector: w4137 -> [w4149 _]
              tunnel: w4148 -> [w4152 w4153]
              tunnel: w4147 -> [w4151 w4168]
              tunnel: w4146 -> [_ w4162]
              tunnel: [w4152 w4161] -> w4145
              tunnel: [w4151 w4160] -> w4144
              tunnel: [UMLEditor_statesType."Idle" ("state") UMLEditor_statesType."Repaint" ("state")] -> w4143
              tunnel: w4141 -> [_ w4156]
              tunnel: w4140 -> [_ w4155]
              tunnel: w4139 -> [_ w4154]
              frame 0, Default {
                n1538 = property on="Diagram" class="Ring (strict)"("Val(Sgnl)"=w4149) -> ()  [unwired: 2 in, 2 out]
              }
              frame -1 {
                n1539 = Strip Path(path=w4154) -> (stripped path=w4164:path, name=w4165:string)
                n1540 = call <resource>:"loadGraph.vi"("filePath"=w4154, "graphics"=w4155, "grid"=w4156, "error in (no error)"=w4153) -> ("reference out"=w4163:refnum<class "Graph.lvclass">, "succeeded"=w4166:bool, "String"=w4159:string, "NodesBounds"=w4157:T10, "error out"=w4167:errorcluster)  [unwired: 11 out]
                n1541 = case shown="True" w4166 {
                  tunnel: w4168 -> [w4170 w4201]
                  tunnel: w4167 -> [_ w4192]
                  tunnel: w4165 -> [_ w4203]
                  tunnel: w4164 -> [_ w4202]
                  tunnel: w4163 -> [_ w4172]
                  tunnel: w4162 -> [_ w4200]
                  tunnel: [w4169 w4180] -> w4161
                  tunnel: w4154 -> [_ w4197]
                  tunnel: [w4170 w4185] -> w4160
                  tunnel: w4159 -> [_ _]
                  tunnel: w4154 -> [_ w4188]
                  tunnel: w4157 -> [_ w4184]
                  tunnel: w4153 -> [w4169 _]
                  frame False {
                  }
                  frame True {
                    w4171 = T1."1" ("GraphButtons")
                    n1542 = case shown="True" w4200 {
                      tunnel: w4192 -> [w4204 w4209]
                      tunnel: [w4205 w4208] -> w4177
                      tunnel: w4201 -> [w4205 w4207]
                      tunnel: [w4204 w4206] -> w4174
                      frame False {
                      }
                      frame True {
                        n1543 = call <resource>:"UMLEditor closeDiagram.vi"("error in (no error)"=w4209, "localVariablesIn"=w4207) -> ("localVariablesOut"=w4208:T5, "error out"=w4206:errorcluster)  [unwired: 16 out]
                      }
                    }
                    n1544 = local write "GraphButtons"(w4171) -> ()
                    n1545 = Bundle By Name(cluster=w4177, "NodesBounds"=w4184, "toolType"=UMLEditor_tooltype."None", "selected"=UMLEditor_tooltype."None" ("selcted")) -> ()  [unwired: 1 out]
                    n1546 = call-dynamic "GetToolbarButtons.vi"("reference"=w4172, "GraphButton"=w4171, "error in (no error)"=w4174) -> ("AllToolbarButtons"=w4176:T36[], "error out"=w4175:errorcluster)  [unwired: 12 in, 3 out]
                    n1547 = Path To String(path=w4188) -> (string=w4189:string)
                    n1548 = call <resource>:"UpdateToolbar.vi"("ToolbarButtons"=w4176, "error in (no error)"=w4175) -> ("error out"=w4173:errorcluster)  [unwired: 17 in]
                    n1549 = property on="Diagram" class="Ring (strict)"("Tip Strip"=w4189) -> ()  [unwired: 2 in, 2 out]
                    n1550 = call <resource>:"UMLEditor addDiagram.vi"("graph"=w4172, "name"=w4203, "saveDir"=w4202, "error in (no error)"=w4173, "localVariablesIn"=w4177) -> ("localVariablesOut"=w4185:T5, "error out"=w4199:errorcluster)  [unwired: 2 in, 11 out]
                    n1551 = Path To String(path=w4197) -> (string=w4196:string)
                    n1552 = Unbundle By Name(w4185) -> ("menu"=w4179:refnum<k9>)
                    n1553 = call <resource>:"UMLEditor menuUpdates.vi"("menu"=w4179, "menuAction"=UMLEditor_MenuActionType."AddRecentFile", "item"=w4196, "addfirst(false)"=TRUE, "error in (no error)"=w4199) -> ("error out"=w4195:errorcluster)  [unwired: 1 in, 13 out]
                    n1554 = call <resource>:"UMLEditor menuUpdates.vi"("menu"=w4179, "menuAction"=UMLEditor_MenuActionType."DiableSave", "error in (no error)"=w4195) -> ("error out"=w4186:errorcluster)  [unwired: 3 in, 13 out]
                    n1555 = property on="GraphButtons" class="RadioBtnsControl (strict)"("Disabled"=u8 0) -> ()  [unwired: 2 in, 2 out]
                    n1556 = property on="Picture" class="Pict"("Visible"=TRUE) -> ()  [unwired: 2 in, 2 out]
                    n1557 = call <resource>:"UMLEditor ToolsMenuUpdates.vi"("menu"=w4179, "Graph"=w4172, "error in (no error)"=w4186) -> ("error out"=w4181:errorcluster)  [unwired: 4 in, 12 out]
                    n1558 = call <resource>:"UndoEngine.vi"("Reference In"=w4172, "Action"=enum16{"TakeSnapshot", "Undo", "Redo"}."TakeSnapshot", "Reset"=TRUE, "error in (no error)"=w4181, "menu"=w4179) -> ("error out"=w4180:errorcluster)  [unwired: 3 in, 11 out]
                  }
                }
              }
            }
          }
        }
        n1559 = local write "Sync"(FALSE ("Sync")) -> ()
        n1560 = call <vilib>:"Unset Busy.vi"("error in (no error)"=w4110) -> ("error out"=w4090:errorcluster)  [unwired: 10 in]
      }
      frame "Close" {
        w4210 = FALSE ("Sync")
        n1561 = call <resource>:"UMLEditor getDiagramInfo.vi"("localVariables"=w4212, "error in (no error)"=w4220) -> ("name"=w4218:string, "unsaved"=w4219:bool, "error out"=w4221:errorcluster)  [unwired: 15 out]
        n1562 = case shown="True" w4219 {
          tunnel: w4218 -> [_ w4268]
          tunnel: [FALSE ("Visible") w4267] -> w4217
          tunnel: w4214 -> [_ w4265]
          tunnel: [_ w4264] -> w4213
          frame False {
          }
          frame True {
            n1563 = Format Into String(format string="SAVE?\nYour work has not been saved!\nDo you want to save: %s", w4268) -> (resulting string=w4266:string)  [unwired: 2 in, 1 out]
            n1564 = case shown="Default" w4265 {
              tunnel: [w4273 w4281] -> w4267
              tunnel: w4266 -> [w4276 w4280]
              tunnel: [w4272 _] -> w4264
              frame "Exit" {
                n1565 = call <vilib>:"Three Button Dialog.vi"("Window Title (\"\")"="Save" ("Window Title (\"\")"), "Right Button Text (\"Cancel\")"="Don't quit" ("F button name (\"Cancel\")"), "Center Button Text (\"No\")"="Don't save" ("F button name (\"Cancel\")"), "Left Button Text (\"Yes\")"="Save" ("T button name (\"OK\")"), "message"=w4276) -> ("Which Button?"=w4271:T32)  [unwired: 6 out]
                n1566 = Greater Or Equal?(x=w4271, y=T32."Right Button") -> (x >= y?=w4272:bool)
                n1567 = Equal?(x=w4271, y=T32."Left Button") -> (x = y?=w4273:bool)
              }
              frame Default {
                n1568 = Two Button Dialog(message=w4280, 1:"Don't save" ("F button name (\"Cancel\")"), 2:"Save" ("T button name (\"OK\")")) -> (T button?=w4281:bool)
              }
            }
          }
        }
        n1569 = local write "Sync"(w4210) -> ()
        n1570 = Bundle By Name(cluster=w4212, "Sync"=w4210) -> (w4211:T5)
        n1571 = case shown="False" w4213 {
          tunnel: [w4228 w4258] -> w4222
          tunnel: w4221 -> [w4227 w4258]
          tunnel: w4217 -> [w4226 _]
          tunnel: [w4225 UMLEditor_statesType."Repaint" ("state")] -> w4216
          tunnel: w4211 -> [w4224 w4260]
          tunnel: [w4223 w4259] -> w4215
          frame False {
            n1572 = case shown="False" w4226 {
              tunnel: [w4240 w4257] -> w4228
              tunnel: w4224 -> [w4238 w4255]
              tunnel: w4227 -> [w4237 w4257]
              tunnel: [w4236 UMLEditor_statesType."Save" ("state")] -> w4225
              tunnel: [w4233 w4255] -> w4223
              frame False {
                n1573 = call <resource>:"UMLEditor closeDiagram.vi"("error in (no error)"=w4237, "localVariablesIn"=w4238) -> ("localVariablesOut"=w4231:T5, "lastDiagramClosed"=w4239:bool, "diagramType"=w4234:T27, "error out"=w4240:errorcluster)  [unwired: 14 out]
                n1574 = Bundle By Name(cluster=w4231, "toolType"=UMLEditor_tooltype."None") -> (w4232:T5)
                n1575 = Unbundle By Name(w4231) -> ("quit"=w4235:bool)
                n1576 = case shown="False" w4235 {
                  tunnel: w4239 -> [w4245 _]
                  tunnel: [w4244 UMLEditor_statesType."Exit" ("state")] -> w4236
                  tunnel: w4234 -> [w4243 _]
                  tunnel: w4232 -> [w4242 w4253]
                  tunnel: [w4241 w4253] -> w4233
                  frame False {
                    n1577 = case shown="False" w4245 {
                      tunnel: [UMLEditor_statesType."Repaint" ("state") UMLEditor_statesType."Idle" ("state")] -> w4244
                      tunnel: w4243 -> [_ _]
                      tunnel: w4242 -> [w4246 w4248]
                      tunnel: [w4246 w4248] -> w4241
                      frame False {
                      }
                      frame True {
                        n1578 = property on="GraphButtons" class="RadioBtnsControl (strict)"("Disabled"=u8 2) -> ()  [unwired: 2 in, 2 out]
                        n1579 = property on="Diagram" class="Ring (strict)"("Strings []"=string[] []) -> ()  [unwired: 2 in, 2 out]
                        n1580 = property on="Picture" class="Pict"("Visible"=FALSE) -> ()  [unwired: 2 in, 2 out]
                      }
                    }
                  }
                  frame True {
                  }
                }
                n1581 = local write "GraphButtons"(T1."1" ("GraphButtons")) -> ()
              }
              frame True {
              }
            }
          }
          frame True {
            n1582 = Bundle By Name(cluster=w4260, "quit"=FALSE) -> (w4259:T5)
          }
        }
      }
      frame "CreateScript" {
        n1583 = Equal?(x=w4303, y=UMLEditor_statesType."ExecuteCommand" ("state")) -> (x = y?=w4286:bool)
        n1584 = call <resource>:"UMLEditor createWizardScriptFile.vi"("localVariables"=w4302, "OnlySelectedNode(False)"=w4286, "error in (no error)"=w4304) -> ("localVariables"=w4301:T5, "error out"=w4284:errorcluster)  [unwired: 15 out]
        n1585 = call <resource>:"CommonVIs_UmlOpenVIRef.vi"("error in"=w4284) -> ("error out"=w4299:errorcluster, "ProjectNameOut"=w4296:string)  [unwired: 3 in, 6 out]
        n1586 = call <resource>:"GDSProject_GetProjects.vi"("GetProjectRefByName"=w4296, "error in (no error)"=w4299) -> ("Projects"=w4298:string[], "Project Refnum"=w4295:refnum<vi>)  [unwired: 1 in, 15 out]
        n1587 = Search 1D Array(1D array=w4298, element=w4296) -> (index of element=w4297:i32)  [unwired: 1 out]
        n1588 = property on="Project" class="Ring (strict)"("Strings []"=w4298, "Value"=w4297) -> ()  [unwired: 2 in, 2 out]
